vi "FuncVI_Sub - VI - Convert CE data to LV data (Variant to Variant).vi"(6 "CE data type":T1=enum."Unknown data type", 7 "LV data (typedef)":variant, 8 "error in":errorcluster, 11 "CE data":variant) -> (0 "error out":errorcluster, 3 "LV data out":variant)   [LabVIEW 2021]
doc: "::: CalcExpress Toolkit :::\nCopyright (c) 2000-2026 Konstantin Shifershteyn. All rights reserved."
uses:
  cetypes.llb/CalcExpress Data Type.ctl
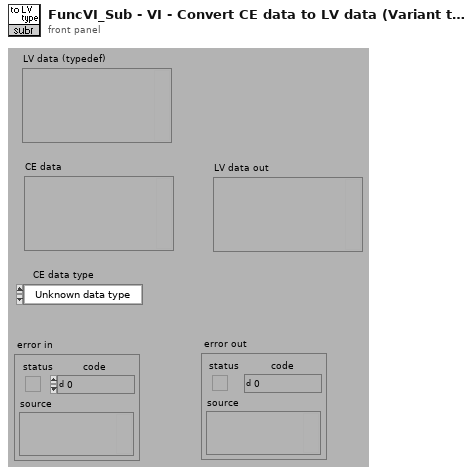
[diagram p1: front panel]
types:
  T1 = typedef "CalcExpress Data Type.ctl" = enum32{"String", "DBL Number", "identifier", "1D Array of DBL", "2D Array of DBL", "CDB Number", "1D Array of CDB", "2D Array of CDB", "1D Array of String", "2D Array of String", "Unknown data type"}
  T2 = enum16{"???", "int8", "int16", "int32", "float32", "float64", "float128", "complex32", "complex64", "complex128", "bool", "string", "path"}
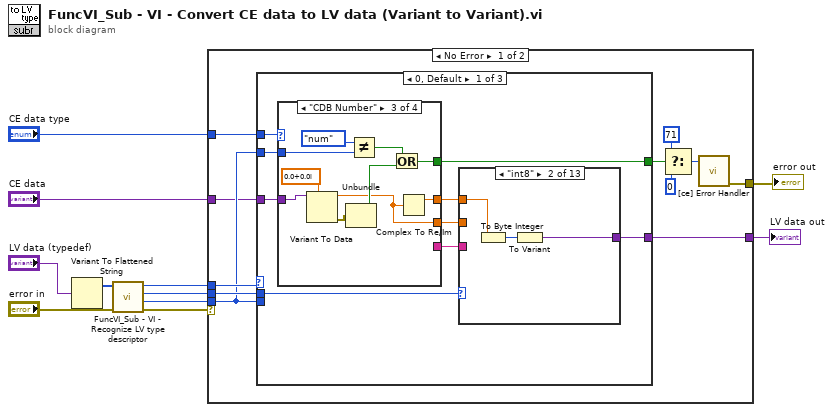
[diagram p0: block diagram]
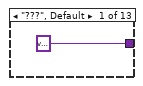
[diagram p2: hidden frame]
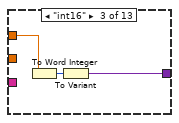
[diagram p3: hidden frame]
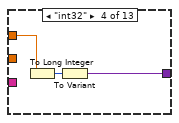
[diagram p4: hidden frame]
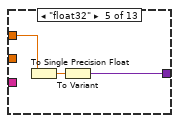
[diagram p5: hidden frame]
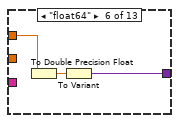
[diagram p6: hidden frame]
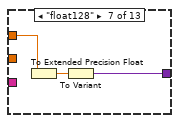
[diagram p7: hidden frame]
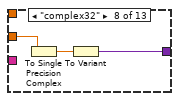
[diagram p8: hidden frame]
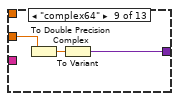
[diagram p9: hidden frame]
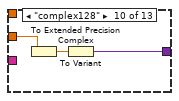
[diagram p10: hidden frame]
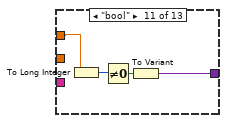
[diagram p11: hidden frame]
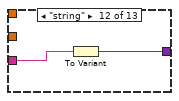
[diagram p12: hidden frame]
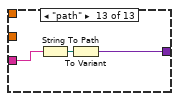
[diagram p13: hidden frame]
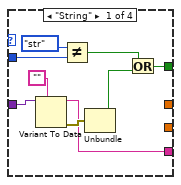
[diagram p14: hidden frame]
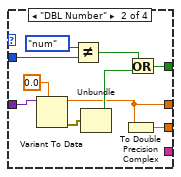
[diagram p15: hidden frame]
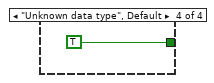
[diagram p16: hidden frame]
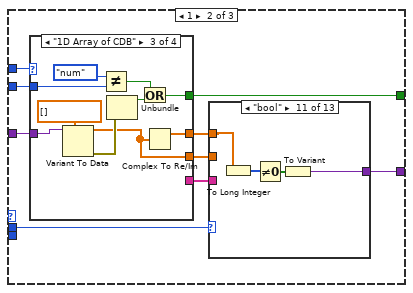
[diagram p17: hidden frame]
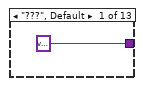
[diagram p18: hidden frame]
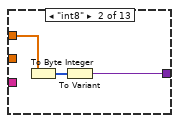
[diagram p19: hidden frame]
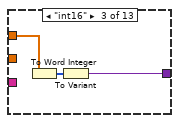
[diagram p20: hidden frame]
diagram:
  n1 = Variant To Flattened String(Variant="LV data (typedef)") -> (1:w2:i16[])  [unwired: 1 out]
  n2 = call "FuncVI_Sub - VI - Recognize LV type descriptor.vi"("error in"="error in", "Type Descriptor"=w2) -> ("error out"=w5:errorcluster, "category"=w7:enum16{"num", "str"}, "representation"=w10:T2, "nDims"=w9:i32)  [unwired: 4 in]
  n3 = case shown="No Error" w5 {
    selector: w5 -> [_ w252]
    tunnel: w10 -> [w22 _]
    tunnel: w9 -> [w21 _]
    tunnel: "CE data type" -> [w20 _]
    tunnel: w7 -> [w17 _]
    tunnel: [w14 w252] -> w6
    tunnel: "CE data" -> [w13 w251]
    tunnel: [w12 w251] -> w1
    frame No Error {
      n4 = case shown="0, Default" w21 {
        tunnel: w22 -> [w29 w103 w179]
        tunnel: w20 -> [w31 w107 w183]
        tunnel: w17 -> [_ _ _]
        tunnel: [w30 w106 w182] -> w16
        tunnel: w17 -> [w27 w105 w181]
        tunnel: w13 -> [w24 w104 w180]
        tunnel: [w23 w99 w175] -> w12
        frame 0, Default {
          n5 = case shown="\"CDB Number\"" w31 {
            tunnel: [w69 _ _ _] -> w25
            tunnel: [_ w78 w97 _] -> w28
            tunnel: [_ w87 w89 _] -> w26
            tunnel: [w73 w84 w92 TRUE ("err")] -> w30
            tunnel: w27 -> [w77 w83 w94 _]
            tunnel: w24 -> [w72 w81 w91 _]
            frame "String" {
              n6 = Variant To Data(type="", Variant=w72) -> (data=w69:string, error out=w71:errorcluster)  [unwired: 1 in]
              n7 = Not Equal?(x=enum16{"num", "str"}."str" ("y"), y=w77) -> (x != y?=w74:bool)
              n8 = Unbundle(w71) -> ("status"=w75:bool)  [unwired: 2 out]
              n9 = Or(x=w74, y=w75) -> (x .or. y?=w73:bool)
            }
            frame "DBL Number" {
              n10 = Variant To Data(type=0.0, Variant=w81) -> (data=w78:dbl, error out=w79:errorcluster)  [unwired: 1 in]
              n11 = Not Equal?(x=enum16{"num", "str"}."num" ("y"), y=w83) -> (x != y?=w85:bool)
              n12 = Unbundle(w79) -> ("status"=w82:bool)  [unwired: 2 out]
              n13 = To Double Precision Complex(1:w78) -> (0:w87:cdb)
              n14 = Or(x=w85, y=w82) -> (x .or. y?=w84:bool)
            }
            frame "CDB Number" {
              n15 = Variant To Data(type=cdb 0.0+0.0i, Variant=w91) -> (data=w89:cdb, error out=w88:errorcluster)  [unwired: 1 in]
              n16 = Unbundle(w88) -> ("status"=w93:bool)  [unwired: 2 out]
              n17 = Not Equal?(x=enum16{"num", "str"}."num" ("y"), y=w94) -> (x != y?=w95:bool)
              n18 = Or(x=w95, y=w93) -> (x .or. y?=w92:bool)
              n19 = Complex To Re/Im(x + iy=w89) -> (x=w97:dbl)  [unwired: 1 out]
            }
            frame "Unknown data type", Default {
            }
          }
          n20 = case shown="\"int8\"" w29 {
            tunnel: w28 -> [_ w35 w38 w41 w44 w47 w50 _ _ _ w63 _ _]
            tunnel: w26 -> [_ _ _ _ _ _ _ w53 w56 w59 _ _ _]
            tunnel: w25 -> [_ _ _ _ _ _ _ _ _ _ _ w65 w68]
            tunnel: [variant ("Variant") w33 w36 w39 w42 w45 w48 w51 w54 w57 w60 w64 w67] -> w23
            frame "???", Default {
            }
            frame "int8" {
              n21 = To Byte Integer(number=w35) -> (8bit integer=w34:i8)
              n22 = To Variant(anything=w34) -> (Variant=w33:variant)
            }
            frame "int16" {
              n23 = To Word Integer(number=w38) -> (16bit integer=w37:i16)
              n24 = To Variant(anything=w37) -> (Variant=w36:variant)
            }
            frame "int32" {
              n25 = To Long Integer(number=w41) -> (32bit integer=w40:i32)
              n26 = To Variant(anything=w40) -> (Variant=w39:variant)
            }
            frame "float32" {
              n27 = To Single Precision Float(number=w44) -> (single precision float=w43:sgl)
              n28 = To Variant(anything=w43) -> (Variant=w42:variant)
            }
            frame "float64" {
              n29 = To Double Precision Float(number=w47) -> (double precision float=w46:dbl)
              n30 = To Variant(anything=w46) -> (Variant=w45:variant)
            }
            frame "float128" {
              n31 = To Extended Precision Float(1:w50) -> (0:w49:ext)
              n32 = To Variant(anything=w49) -> (Variant=w48:variant)
            }
            frame "complex32" {
              n33 = To Single Precision Complex(1:w53) -> (0:w52:csg)
              n34 = To Variant(anything=w52) -> (Variant=w51:variant)
            }
            frame "complex64" {
              n35 = To Double Precision Complex(1:w56) -> (0:w55:cdb)
              n36 = To Variant(anything=w55) -> (Variant=w54:variant)
            }
            frame "complex128" {
              n37 = To Extended Precision Complex(1:w59) -> (0:w58:cxt)
              n38 = To Variant(anything=w58) -> (Variant=w57:variant)
            }
            frame "bool" {
              n39 = To Long Integer(number=w63) -> (32bit integer=w62:i32)
              n40 = Not Equal To 0?(x=w62) -> (x != 0?=w61:bool)
              n41 = To Variant(anything=w61) -> (Variant=w60:variant)
            }
            frame "string" {
              n42 = To Variant(anything=w65) -> (Variant=w64:variant)
            }
            frame "path" {
              n43 = String To Path(string=w68) -> (path=w66:path)
              n44 = To Variant(anything=w66) -> (Variant=w67:variant)
            }
          }
        }
        frame 1 {
          n45 = case shown="\"1D Array of CDB\"" w107 {
            tunnel: [w145 _ _ _] -> w102
            tunnel: [_ w154 w173 _] -> w100
            tunnel: [_ w163 w164 _] -> w101
            tunnel: [w149 w160 w168 TRUE ("err")] -> w106
            tunnel: w105 -> [w153 w159 w170 _]
            tunnel: w104 -> [w148 w157 w167 _]
            frame "1D Array of String" {
              n46 = Variant To Data(type=string[] [], Variant=w148) -> (data=w145:string[], error out=w146:errorcluster)  [unwired: 1 in]
              n47 = Unbundle(w146) -> ("status"=w151:bool)  [unwired: 2 out]
              n48 = Not Equal?(x=enum16{"num", "str"}."str" ("y"), y=w153) -> (x != y?=w150:bool)
              n49 = Or(x=w150, y=w151) -> (x .or. y?=w149:bool)
            }
            frame "1D Array of DBL" {
              n50 = Variant To Data(type=dbl[] [], Variant=w157) -> (data=w154:dbl[], error out=w155:errorcluster)  [unwired: 1 in]
              n51 = Not Equal?(x=enum16{"num", "str"}."num" ("y"), y=w159) -> (x != y?=w161:bool)
              n52 = Unbundle(w155) -> ("status"=w158:bool)  [unwired: 2 out]
              n53 = To Double Precision Complex(1:w154) -> (0:w163:cdb[])
              n54 = Or(x=w161, y=w158) -> (x .or. y?=w160:bool)
            }
            frame "1D Array of CDB" {
              n55 = Variant To Data(type=cdb[] [], Variant=w167) -> (data=w164:cdb[], error out=w166:errorcluster)  [unwired: 1 in]
              n56 = Not Equal?(x=enum16{"num", "str"}."num" ("y"), y=w170) -> (x != y?=w171:bool)
              n57 = Unbundle(w166) -> ("status"=w169:bool)  [unwired: 2 out]
              n58 = Or(x=w171, y=w169) -> (x .or. y?=w168:bool)
              n59 = Complex To Re/Im(x + iy=w164) -> (x=w173:dbl[])  [unwired: 1 out]
            }
            frame "Unknown data type", Default {
            }
          }
          n60 = case shown="\"bool\"" w103 {
            tunnel: w100 -> [_ w111 w114 w117 w120 w123 w126 _ _ _ w139 _ _]
            tunnel: w101 -> [_ _ _ _ _ _ _ w129 w132 w135 _ _ _]
            tunnel: w102 -> [_ _ _ _ _ _ _ _ _ _ _ w141 w144]
            tunnel: [variant ("Variant") w109 w112 w115 w118 w121 w124 w127 w130 w133 w136 w140 w143] -> w99
            frame "???", Default {
            }
            frame "int8" {
              n61 = To Byte Integer(number=w111) -> (8bit integer=w110:i8[])
              n62 = To Variant(anything=w110) -> (Variant=w109:variant)
            }
            frame "int16" {
              n63 = To Word Integer(number=w114) -> (16bit integer=w113:i16[])
              n64 = To Variant(anything=w113) -> (Variant=w112:variant)
            }
            frame "int32" {
              n65 = To Long Integer(number=w117) -> (32bit integer=w116:i32[])
              n66 = To Variant(anything=w116) -> (Variant=w115:variant)
            }
            frame "float32" {
              n67 = To Single Precision Float(number=w120) -> (single precision float=w119:sgl[])
              n68 = To Variant(anything=w119) -> (Variant=w118:variant)
            }
            frame "float64" {
              n69 = To Double Precision Float(number=w123) -> (double precision float=w122:dbl[])
              n70 = To Variant(anything=w122) -> (Variant=w121:variant)
            }
            frame "float128" {
              n71 = To Extended Precision Float(1:w126) -> (0:w125:ext[])
              n72 = To Variant(anything=w125) -> (Variant=w124:variant)
            }
            frame "complex32" {
              n73 = To Single Precision Complex(1:w129) -> (0:w128:csg[])
              n74 = To Variant(anything=w128) -> (Variant=w127:variant)
            }
            frame "complex64" {
              n75 = To Double Precision Complex(1:w132) -> (0:w131:cdb[])
              n76 = To Variant(anything=w131) -> (Variant=w130:variant)
            }
            frame "complex128" {
              n77 = To Extended Precision Complex(1:w135) -> (0:w134:cxt[])
              n78 = To Variant(anything=w134) -> (Variant=w133:variant)
            }
            frame "bool" {
              n79 = To Long Integer(number=w139) -> (32bit integer=w138:i32[])
              n80 = Not Equal To 0?(x=w138) -> (x != 0?=w137:bool[])
              n81 = To Variant(anything=w137) -> (Variant=w136:variant)
            }
            frame "string" {
              n82 = To Variant(anything=w141) -> (Variant=w140:variant)
            }
            frame "path" {
              n83 = String To Path(string=w144) -> (path=w142:path[])
              n84 = To Variant(anything=w142) -> (Variant=w143:variant)
            }
          }
        }
        frame 2 {
          n85 = case shown="\"2D Array of CDB\"" w183 {
            tunnel: [w221 _ _ _] -> w178
            tunnel: [_ w230 w249 _] -> w176
            tunnel: [_ w239 w240 _] -> w177
            tunnel: [w225 w236 w244 TRUE ("err")] -> w182
            tunnel: w181 -> [w229 w235 w246 _]
            tunnel: w180 -> [w224 w233 w243 _]
            frame "2D Array of String" {
              n86 = Variant To Data(type=string[][] [], Variant=w224) -> (data=w221:string[][], error out=w223:errorcluster)  [unwired: 1 in]
              n87 = Unbundle(w223) -> ("status"=w227:bool)  [unwired: 2 out]
              n88 = Not Equal?(x=enum16{"num", "str"}."str" ("y"), y=w229) -> (x != y?=w226:bool)
              n89 = Or(x=w226, y=w227) -> (x .or. y?=w225:bool)
            }
            frame "2D Array of DBL" {
              n90 = Variant To Data(type=dbl[][] [], Variant=w233) -> (data=w230:dbl[][], error out=w232:errorcluster)  [unwired: 1 in]
              n91 = Not Equal?(x=enum16{"num", "str"}."num" ("y"), y=w235) -> (x != y?=w237:bool)
              n92 = Unbundle(w232) -> ("status"=w234:bool)  [unwired: 2 out]
              n93 = To Double Precision Complex(1:w230) -> (0:w239:cdb[][])
              n94 = Or(x=w237, y=w234) -> (x .or. y?=w236:bool)
            }
            frame "2D Array of CDB" {
              n95 = Variant To Data(type=cdb[][] [], Variant=w243) -> (data=w240:cdb[][], error out=w241:errorcluster)  [unwired: 1 in]
              n96 = Not Equal?(x=enum16{"num", "str"}."num" ("y"), y=w246) -> (x != y?=w247:bool)
              n97 = Unbundle(w241) -> ("status"=w245:bool)  [unwired: 2 out]
              n98 = Complex To Re/Im(x + iy=w240) -> (x=w249:dbl[][])  [unwired: 1 out]
              n99 = Or(x=w247, y=w245) -> (x .or. y?=w244:bool)
            }
            frame "Unknown data type", Default {
            }
          }
          n100 = case shown="\"bool\"" w179 {
            tunnel: w176 -> [_ w187 w190 w193 w196 w199 w202 _ _ _ w215 _ _]
            tunnel: w177 -> [_ _ _ _ _ _ _ w205 w208 w211 _ _ _]
            tunnel: w178 -> [_ _ _ _ _ _ _ _ _ _ _ w217 w220]
            tunnel: [variant ("Variant") w185 w188 w191 w194 w197 w200 w203 w206 w209 w212 w216 w219] -> w175
            frame "???", Default {
            }
            frame "int8" {
              n101 = To Byte Integer(number=w187) -> (8bit integer=w186:i8[][])
              n102 = To Variant(anything=w186) -> (Variant=w185:variant)
            }
            frame "int16" {
              n103 = To Word Integer(number=w190) -> (16bit integer=w189:i16[][])
              n104 = To Variant(anything=w189) -> (Variant=w188:variant)
            }
            frame "int32" {
              n105 = To Long Integer(number=w193) -> (32bit integer=w192:i32[][])
              n106 = To Variant(anything=w192) -> (Variant=w191:variant)
            }
            frame "float32" {
              n107 = To Single Precision Float(number=w196) -> (single precision float=w195:sgl[][])
              n108 = To Variant(anything=w195) -> (Variant=w194:variant)
            }
            frame "float64" {
              n109 = To Double Precision Float(number=w199) -> (double precision float=w198:dbl[][])
              n110 = To Variant(anything=w198) -> (Variant=w197:variant)
            }
            frame "float128" {
              n111 = To Extended Precision Float(1:w202) -> (0:w201:ext[][])
              n112 = To Variant(anything=w201) -> (Variant=w200:variant)
            }
            frame "complex32" {
              n113 = To Single Precision Complex(1:w205) -> (0:w204:csg[][])
              n114 = To Variant(anything=w204) -> (Variant=w203:variant)
            }
            frame "complex64" {
              n115 = To Double Precision Complex(1:w208) -> (0:w207:cdb[][])
              n116 = To Variant(anything=w207) -> (Variant=w206:variant)
            }
            frame "complex128" {
              n117 = To Extended Precision Complex(1:w211) -> (0:w210:cxt[][])
              n118 = To Variant(anything=w210) -> (Variant=w209:variant)
            }
            frame "bool" {
              n119 = To Long Integer(number=w215) -> (32bit integer=w214:i32[][])
              n120 = Not Equal To 0?(x=w214) -> (x != 0?=w213:bool[][])
              n121 = To Variant(anything=w213) -> (Variant=w212:variant)
            }
            frame "string" {
              n122 = To Variant(anything=w217) -> (Variant=w216:variant)
            }
            frame "path" {
              n123 = String To Path(string=w220) -> (path=w218:path[][])
              n124 = To Variant(anything=w218) -> (Variant=w219:variant)
            }
          }
        }
      }
      n125 = Select(t=71, s=w16, f=0) -> (s? t:f=w15:i32)
      n126 = call "[ce] Error Handler.vi"("error code"=w15) -> ("error out"=w14:errorcluster)  [unwired: 9 in, 1 out]
    }
    frame Error {
    }
  }
  "error out" <- w6
  "LV data out" <- w1
